vi "ACTIVIDAD INSERT INTO ARRAY.vi"() -> ()   [LabVIEW 2026]
panel:
  in  "ARREGLO ORIGINAL":dbl[](array[numeric])
  out "INDICADOR NÚMERO AGREGADO":i32[](array[numeric])
  in  "NÚMERO A AGREGAR":dbl
  in  "INDICE":i16
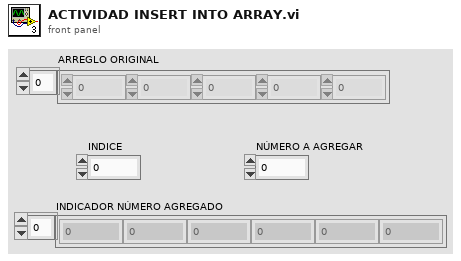
[diagram p1: front panel]
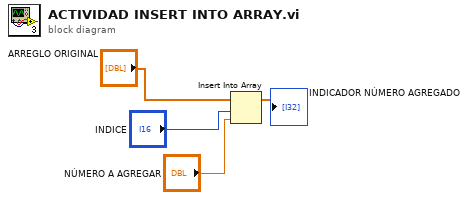
[diagram p0: block diagram]
diagram:
  n1 = Insert Into Array(array="ARREGLO ORIGINAL", index="INDICE", new element="NÚMERO A AGREGAR") -> (→"INDICADOR NÚMERO AGREGADO":dbl[])
